vi "RemoteVI Complex Fixture Children.vi"(0 "Control":refnum<vi>, 11 "error in":errorcluster) -> (4 "Children":refnum<vi>[](array[refnum]), 15 "error out":errorcluster)   [LabVIEW 2020]
doc: "Helper of RemoteVI Complex Fixture.vi. Returns the controls one level inside Control: the controls on every page of a tab control, the elements of a cluster, nothing for any other control. Errors of the casts are not errors here (a control that is neither is the normal case); errors of the property reads go to error out."
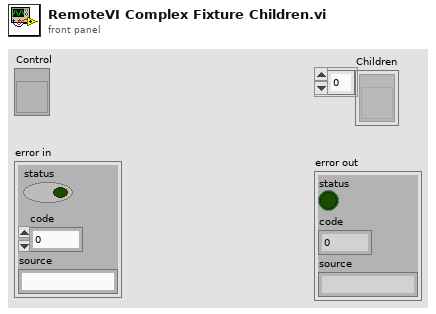
[diagram p1: front panel]
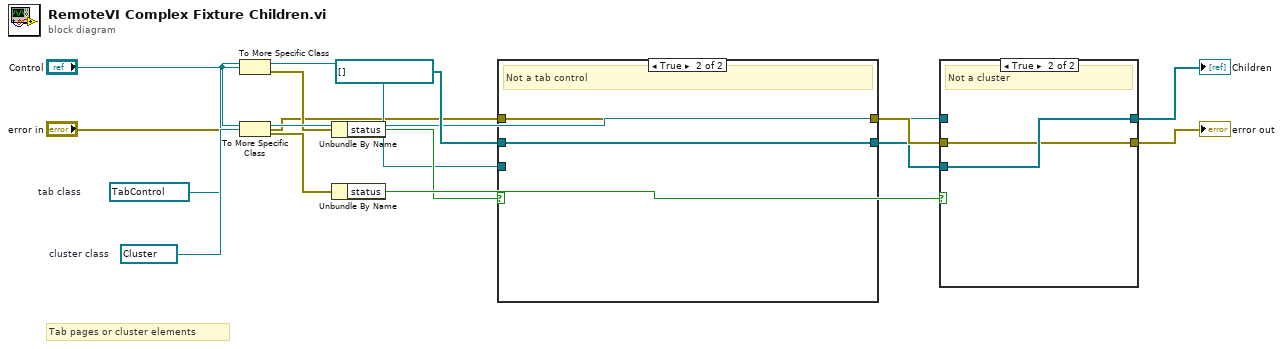
[diagram p0: block diagram]
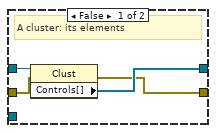
[diagram p2: hidden frame]
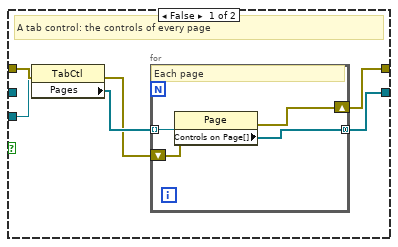
[diagram p3: hidden frame]
diagram:
  w4 = refnum<vi> refnum  # cluster class
  w3 = refnum<vi> refnum  # tab class
  # "Tab pages or cluster elements"
  n1 = To More Specific Class(target class=w3, reference="Control") -> (specific class reference=w5:refnum<vi>, error out=w6:errorcluster)  [unwired: 1 in]
  n2 = To More Specific Class(target class=w4, reference="Control") -> (specific class reference=w7:refnum<vi>, error out=w8:errorcluster)  [unwired: 1 in]
  n3 = Unbundle By Name(w6) -> ("status"=w9:bool)
  n4 = Unbundle By Name(w8) -> ("status"=w10:bool)
  n5 = case shown="True" w9 {
    tunnel: "error in" -> [w17 w26]
    tunnel: refnum<vi>[] [] -> [_ w27]
    tunnel: w5 -> [w16 _]
    tunnel: [w20 w26] -> w13
    tunnel: [w21 w27] -> w12
    frame False {
      # "A tab control: the controls of every page"
      n6 = property class="TabCtl"(reference=w16, error in=w17) -> (error out=w18:errorcluster, "Pages"=w19:refnum<vi>[])  [unwired: 1 out]
      n7 = for {
        tunnel: w19 -> [w22] mode=indexing
        shift-right: [w24] -> w20
        shift-left: w18 -> [w23]
        tunnel: [w25] -> w21 mode=concatenating
        # "Each page"
        n8 = property class="Page"(reference=w22, error in=w23) -> (error out=w24:errorcluster, "Controls on Page[]"=w25:refnum<vi>[])  [unwired: 1 out]
      }
    }
    frame True {
      # "Not a tab control"
    }
  }
  n9 = case shown="True" w10 {
    tunnel: w7 -> [w28 _]
    tunnel: w13 -> [w29 w32]
    tunnel: w12 -> [_ w33]
    tunnel: [w31 w33] -> w14
    tunnel: [w30 w32] -> w15
    frame False {
      # "A cluster: its elements"
      n10 = property class="Clust"(reference=w28, error in=w29) -> (error out=w30:errorcluster, "Controls[]"=w31:refnum<vi>[])  [unwired: 1 out]
    }
    frame True {
      # "Not a cluster"
    }
  }
  "Children" <- w14
  "error out" <- w15
